vi "set Marker Peak Search Type.vi"(8 "error in (no error)":errorcluster, 9 "Marker Index":i32, 10 "Peak Search Type":T1, 11 "FSV-40N in":refnum<class "FSV-40N.lvclass">) -> (0 "error out":errorcluster, 3 "FSV-40N out":refnum<class "FSV-40N.lvclass">)   [LabVIEW 2023, in "Spectrum Analyzer.lvlib" / "FSV-40N.lvclass"]
uses:
  FSV-40N.lvclass
  TYPE DEFINITION/TYPE Marker Peak Search Type.ctl
  TYPE DEFINITION/TYPE Marker Control Mode.ctl
  FSV-40N.lvclass/FSV-40N.ctl
  <vilib>/ErrorRing/Error Ring.xnode
  Spectrum Analyzer.lvlib
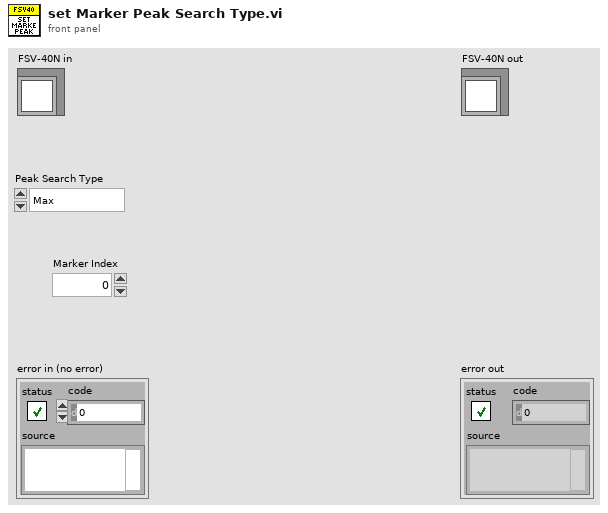
[diagram p1: front panel]
types:
  T1 = typedef "Spectrum Analyzer.lvlib/TYPE Marker Peak Search Type.ctl" = enum16{"Max", "Next Peak", "Max - Auto"}
  T2 = typedef "Spectrum Analyzer.lvlib/TYPE Marker Control Mode.ctl" = enum16{"Normal", "Delta", "Off"}
  T3 = typedef "Spectrum Analyzer.lvlib/TYPE Marker Type Map.ctl" = map{i32, T2}
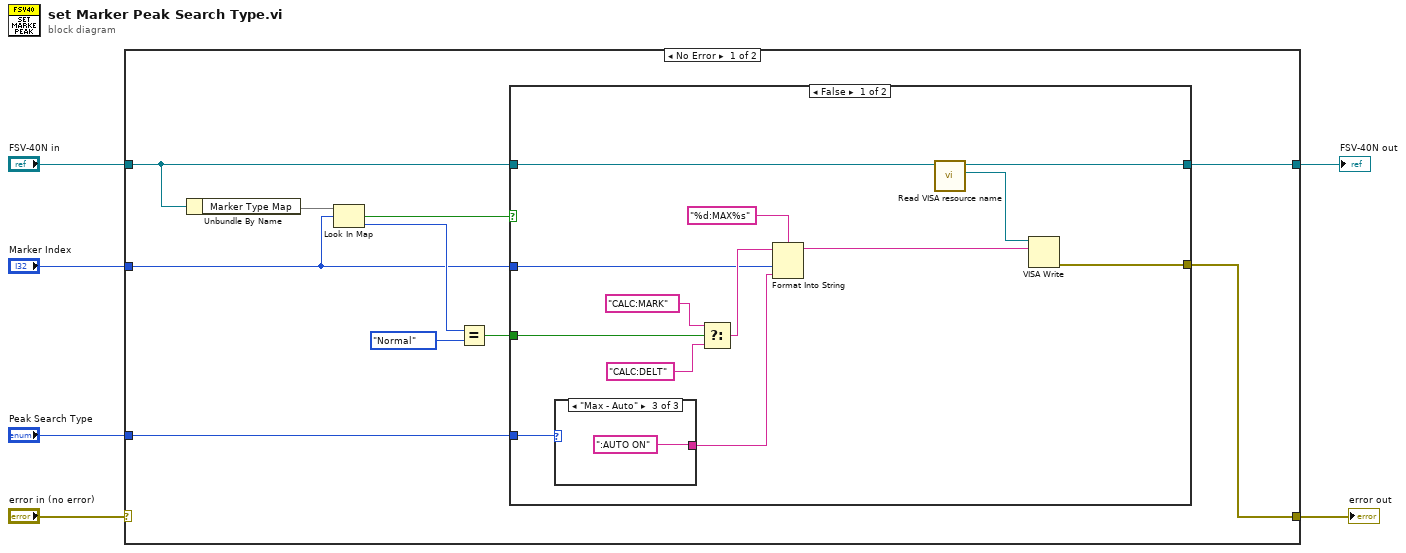
[diagram p0: block diagram]
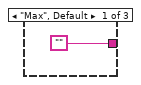
[diagram p2: hidden frame]
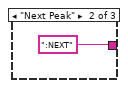
[diagram p3: hidden frame]
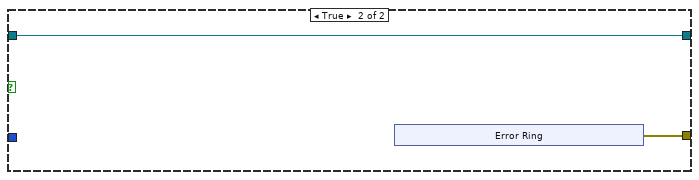
[diagram p4: hidden frame]
diagram:
  n1 = case shown="No Error" "error in (no error)" {
    selector: "error in (no error)" -> [_ w36]
    tunnel: "FSV-40N in" -> [w12 w37]
    tunnel: [w15 w37] -> w5
    tunnel: [w16 w36] -> w3
    tunnel: "Marker Index" -> [w7 _]
    tunnel: "Peak Search Type" -> [w8 _]
    frame No Error {
      n2 = Unbundle By Name(w12) -> ("Marker Type Map"=w11:T3)
      n3 = Look In Map(map=w11, key=w7) -> (key not found?=w9:bool, value=w10:T2)  [unwired: 1 in]
      n4 = Equal?(x=w10, y=TYPE_Marker_Control_Mode."Normal") -> (x = y?=w13:bool)
      n5 = case shown="False" w9 {
        tunnel: [w28 w33] -> w16
        tunnel: [w27 w34] -> w15
        tunnel: w13 -> [w26 _]
        tunnel: w12 -> [w22 w34]
        tunnel: w8 -> [w20 _]
        tunnel: w7 -> [w21 _]
        frame False {
          n6 = case shown="\"Max - Auto\"" w20 {
            tunnel: ["" ":NEXT" ":AUTO ON"] -> w19
            frame "Max", Default {
            }
            frame "Next Peak" {
            }
            frame "Max - Auto" {
            }
          }
          n7 = Select(t="CALC:MARK" ("initial string"), s=w26, f="CALC:DELT" ("initial string")) -> (s? t:f=w23:string)
          n8 = Format Into String(format string="%d:MAX%s", initial string=w23, w21, w19) -> (resulting string=w18:string)  [unwired: 1 in, 1 out]
          n9 = call "Read VISA resource name.vi"("FSV-40N in"=w22) -> ("VISA resource name"=w17:refnum<visa-resource-name>, "FSV-40N out"=w27:refnum<class "FSV-40N.lvclass">)  [unwired: 8 in, 1 out]
          n10 = VISA Write(VISA resource name=w17, write buffer=w18) -> (error out=w28:errorcluster)  [unwired: 1 in, 2 out]
        }
        frame True {
          n11 = xnode "Error Ring"() -> ("error out"=w33:errorcluster)
        }
      }
    }
    frame Error {
    }
  }
  "error out" <- w3
  "FSV-40N out" <- w5
